vi "VIH HelpGen - Image - Make Control Name Picture.vi"(9 "Wire Rule":T1(ring), 11 "Control name":string) -> (3 "Image 2D Array":u32[][](array[numeric]) format="%.0x")   [LabVIEW 2014]
doc: "::: VI Helpeks :::\nCopyright (c) 2000-2026 Konstantin Shifershteyn. All rights reserved."
panel:
  # "VI Helpeks\nCopyright (c) 2012-2026 Konstantin Shifershteyn"
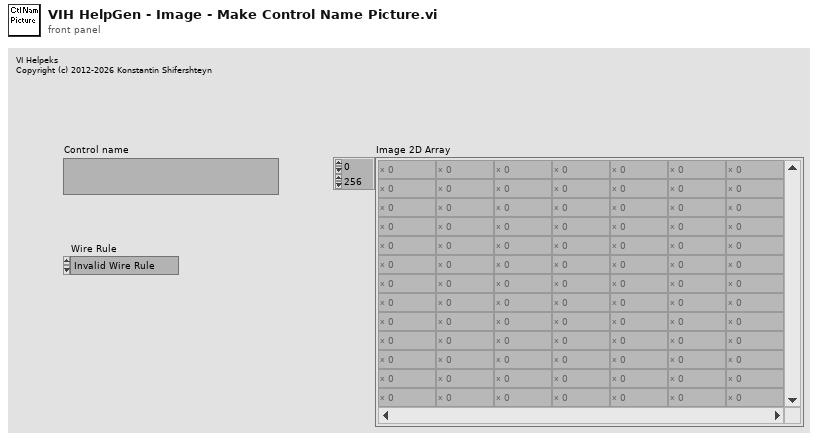
[diagram p1: front panel]
types:
  T1 = enum16{"Invalid Wire Rule", "Required", "Recommended", "Optional", "Dynamic Dispatch"}
  T2 = enum16{"User-specified Font", "Application Font", "System Font", "Dialog Font"}
  T3 = cluster{"Font Name:":string, "Size":i16, "Strikeout?":bool, "Italic?":bool, "Underline?":bool, "Outline?":bool, "Shadow?":bool, "Bold?":bool}
  T4 = typedef "imagedata.ctl" = cluster{"image type":i32, "image depth":i32, "image":u8[], "mask":u8[], "colors":u32[], "Rectangle":cluster{"left":i16, "top":i16, "right":i16, "bottom":i16}}
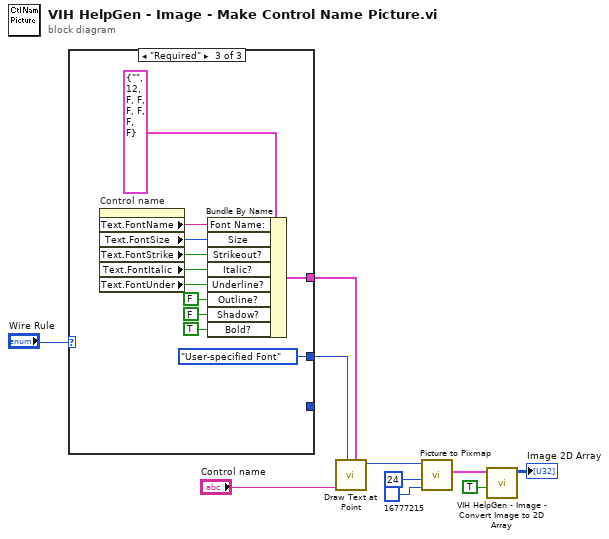
[diagram p0: block diagram]
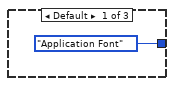
[diagram p2: hidden frame]
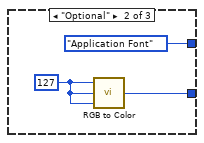
[diagram p3: hidden frame]
diagram:
  n1 = case shown="\"Required\"" "Wire Rule" {
    tunnel: [T2."Application Font" ("desired font(Application)") T2."Application Font" ("desired font(Application)") T2."User-specified Font" ("desired font(Application)")] -> w6
    tunnel: [_ _ w15] -> w4
    tunnel: [_ w12 _] -> _
    frame Default {
    }
    frame "Optional" {
      w13 = u8 127 ("R")
      n2 = call <vilib>:"RGB to Color.vi"("B"=w13, "G"=w13, "R"=w13) -> ("Color"=w12:u32)
    }
    frame "Required" {
      n3 = property on="Control name" class="Str"() -> ("Text.FontName"=w24:string, "Text.FontSize"=w23:u32, "Text.FontStrike"=w22:bool, "Text.FontItalic"=w21:bool, "Text.FontUnder"=w20:bool)  [unwired: 2 in, 2 out]
      n4 = Bundle By Name(cluster=T3 {"Font Name:"="", "Size"=12, "Strikeout?"=FALSE, "Italic?"=FALSE, "Underline?"=FALSE, "Outline?"=FALSE, "Shadow?"=FALSE, "Bold?"=FALSE} ("[user-specified font]"), "Font Name:"=w24, "Size"=w23, "Strikeout?"=w22, "Italic?"=w21, "Underline?"=w20, "Outline?"=FALSE, "Shadow?"=FALSE, "Bold?"=TRUE) -> (w15:T3)
    }
  }
  n5 = call <vilib>:"Draw Text at Point.vi"("[user-specified font]"=w4, "desired font(Application)"=w6, "text"="Control name") -> ("new picture"=w9:picture)  [unwired: 7 in, 1 out]
  n6 = call <vilib>:"Picture to Pixmap.vi"("Background Color"=u32 16777215, "depth"=24, "picture"=w9) -> ("image data"=w10:T4)  [unwired: 7 in, 1 out]
  n7 = call "VIH HelpGen - Image - Convert Image to 2D Array.vi"("Black & White (F)"=TRUE, "Image Data"=w10) -> ("Image 2D Array"=→"Image 2D Array":u32[][])  [unwired: 7 in, 2 out]
